vi "get UI reference.vi"(8 "error in":errorcluster, 11 "protection settings in":refnum<class "protection settings.lvclass">) -> (0 "error out":errorcluster, 2 "VI Refnum":refnum<vi>, 3 "protection settings out":refnum<class "protection settings.lvclass">)   [LabVIEW 2013, in "protection settings.lvclass"]
uses:
  protection settings.lvclass
  protect ui.vi
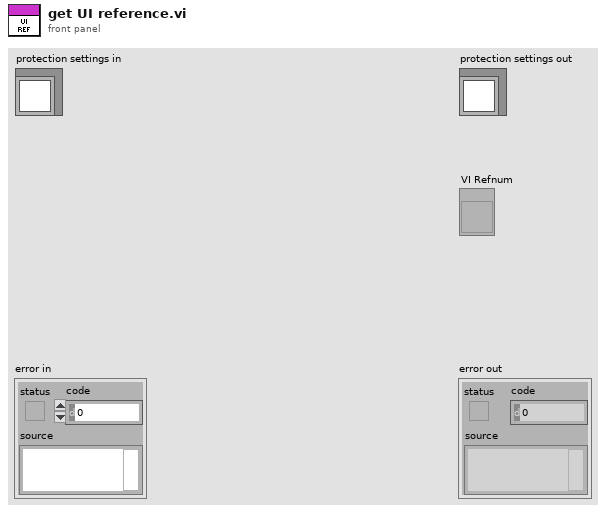
[diagram p1: front panel]
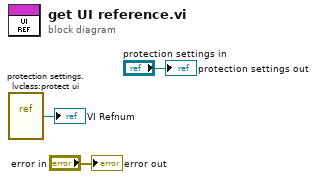
[diagram p0: block diagram]
diagram:
  n1 = vi-ref "protection settings.lvclass:protect ui.vi"() -> (→"VI Refnum":refnum<vi>)
  "error out" <- "error in"
  "protection settings out" <- "protection settings in"
